vi "Mise_en_forme_programme EPC.vi"(1 "Programme en entrée":cluster{"String":string, "value":dbl}[](array[cluster]) {"value" format="%#.1f"}) -> (0 "Programme en sortie":cluster{string, dbl}[][](array[cluster]) {"?" format="%#.1f"})   [LabVIEW 2022 SP3]
panel:
  out "Nb segments":i32
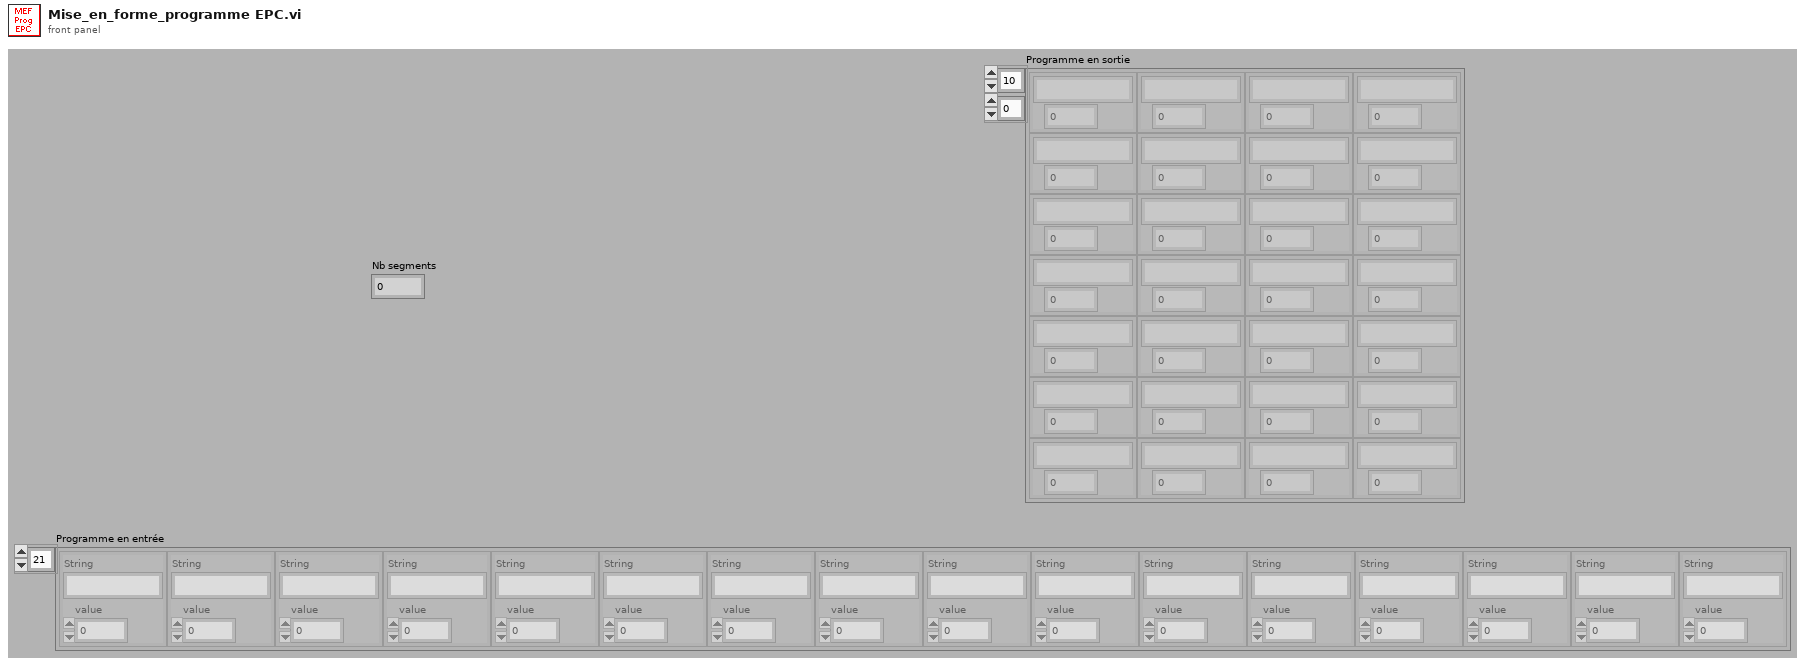
[diagram p1: front panel]
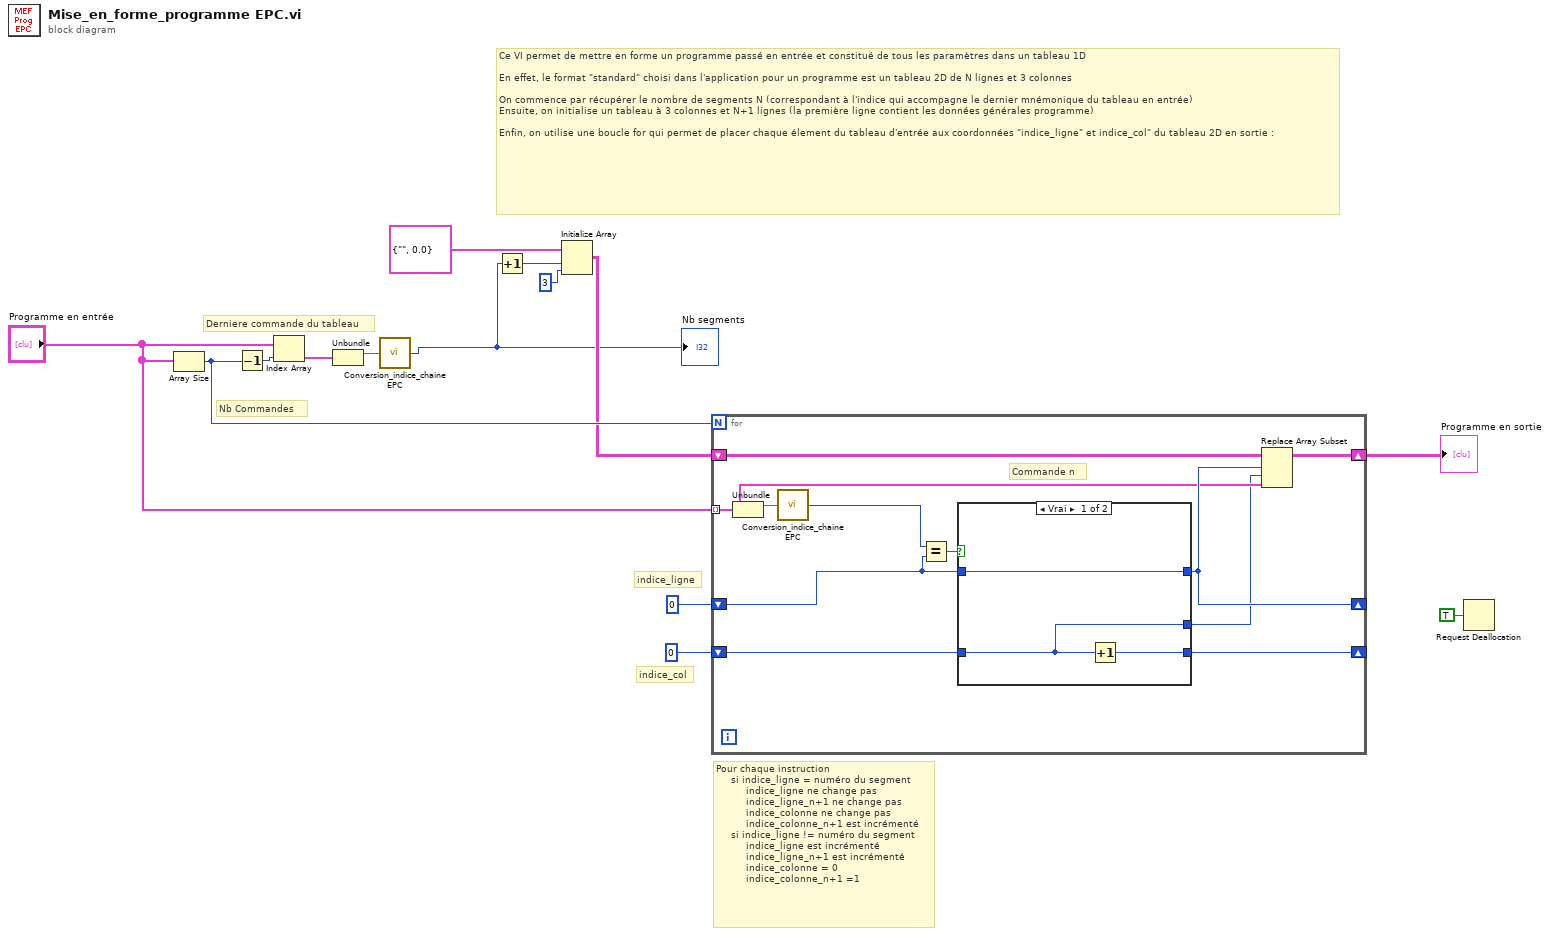
[diagram p0: block diagram]
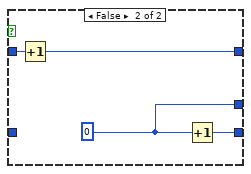
[diagram p2: hidden frame]
diagram:
  # "Pour chaque instruction\n     si indice_ligne = numéro du segment\n          indice_ligne ne change pas\n          indice_ligne_n+1 ne change pas\n          indice_colonne ne change pas\n          indice_colonne_n+1 est incrémenté\n     si indice_ligne != numéro du segment\n          indice_ligne est incrémenté\n          indice_ligne_n+1 est incrémenté\n          indice_colonne = 0\n          indice_colonne_n+1 =1"
  # "Ce VI permet de mettre en forme un programme passé en entrée et constitué de tous les paramètres dans un tableau 1D\n\nEn effet, le format \"standard\" choisi dans l'application pour un programme est un tableau 2D de N lignes et 3 colonnes\n\nOn commence par récupérer le nombre de segments N (correspondant à l'indice qui accompagne le dernier mnémonique du tableau en entrée)\nEnsuite, on initialise un tableau à 3 colonnes et N+1 lignes (la première ligne contient les données générales programme)\n\nEnfin, on utilise une boucle for qui permet de placer chaque élement du tableau d'entrée aux coordonnées \"indice_ligne\" et indice_col\" du tableau 2D en sortie :"
  # "indice_ligne"
  # "indice_col"
  # "Nb Commandes"
  # "Derniere commande du tableau"
  n1 = Array Size(array="Programme en entrée") -> (size(s)=w10:i32)
  n2 = Decrement(x=w10) -> (x-1=w14:i32)
  n3 = Index Array(array="Programme en entrée", index=w14) -> (element=w13:cluster{"String":string, "value":dbl})
  n4 = Unbundle(w13) -> ("String"=w2:string)  [unwired: 1 out]
  n5 = call "Conversion_indice_chaine EPC.vi"("Chaîne indice"=w2) -> ("Indice"=w1:i32)
  "Nb segments" <- w1
  n6 = Increment(x=w1) -> (x+1=w6:i32)
  n7 = Initialize Array(cluster{string, dbl} {"", 0.0}, w6, 3 ("taille de la dimension")) -> (w5:cluster{string, dbl}[][])
  n8 = for {
    N: w10 -> [_]
    tunnel: "Programme en entrée" -> [w19] mode=indexing
    shift-right: [w18] -> _
    shift-left: 0 -> [w24]
    shift-right: [w20] -> _
    shift-left: 0 -> [w23]
    shift-right: [w21] -> w4
    shift-left: w5 -> [w22]
    # "Commande n"
    n9 = Unbundle(w19) -> ("String"=w16:string)  [unwired: 1 out]
    n10 = call "Conversion_indice_chaine EPC.vi"("Chaîne indice"=w16) -> ("Indice"=w15:i32)
    n11 = Equal?(x=w15, y=w23) -> (x = y?=w25:bool)
    n12 = case shown="Vrai" w25 {
      tunnel: w24 -> [w26 _]
      tunnel: [w28 w30] -> w18
      tunnel: w23 -> [w27 w32]
      tunnel: [w27 w31] -> w20
      tunnel: [w26 w29] -> w17
      frame True {
        n13 = Increment(x=w26) -> (x+1=w28:i32)
      }
      frame False {
        w29 = 0
        n14 = Increment(x=w32) -> (x+1=w31:i32)
        n15 = Increment(x=w29) -> (x+1=w30:i32)
      }
    }
    n16 = Replace Array Subset(array=w22, new element=w19, index (row)=w20, index (col)=w17) -> (w21:cluster{string, dbl}[][])
  }
  "Programme en sortie" <- w4
  n17 = Request Deallocation(TRUE ("flag")) -> ()
